vi "labview-quick-extractor.vi"   [LabVIEW 2020]
uses:
  Nominal Client/Nominal Client.lvclass/Nominal Client.ctl
  User/User.lvclass
  Nominal Client/Nominal Client.lvclass
  nominal types/workspace/workspace.lvclass
  submodules/reqwest-labview/lv-src/reqwest/reqwest.lvclass
  datasources/s3/s3.lvclass
  C:/sw/labview-client/lv_src/datasources/source/source.lvclass
  C:/sw/labview-client/lv_src/datasources/payload/payload.lvclass
  C:/sw/labview-client/lv_src/datasources/s3/s3.lvclass
  e79185ee-863a-4b48-b269-365b27d9e424.vi
  Nominal Client/ingest_containerized.vi
  Nominal Client/catalog.wait_until_multiple_ingest_complete.vi
  datasources/target/target.lvclass
  datasources/target/create_new.vi
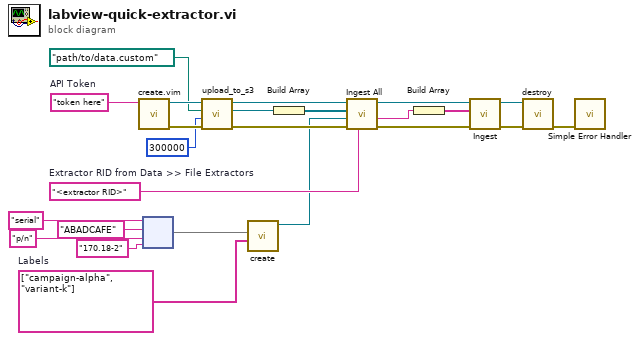
[diagram p0: block diagram]
diagram:
  w2 = string[] ["campaign-alpha", "variant-k"]  # Labels
  w8 = "<extractor RID>"  # Extractor RID from Data >> File Extractors
  w23 = "token here"  # API Token
  n1 = call "create.vim"("API Token (string or path)"=w23) -> ("error out"=w21:errorcluster, "Nominal Client"=w22:refnum<class "Nominal Client.lvclass">)  [unwired: 8 in, 1 out]
  n2 = node("serial", "ABADCAFE", "p/n", "170.18-2") -> (w3:map{string, string})
  n3 = call "upload_to_s3.vi"("error in"=w21, "timeout per chunk (ms)"=300000 ("timeout (ms)"), "File"=path "path/to/data.custom" ("File Path"), "Nominal Client in"=w22) -> ("error out"=w17:errorcluster, "source"=w16:refnum<class "s3.lvclass">, "Nominal Client out"=w18:refnum<class "Nominal Client.lvclass">)  [unwired: 5 in]
  n4 = call-poly "create.vi"("Labels"=w2, "Properties"=w3) -> ("New Target"=w1:refnum<class "target.lvclass">)  [unwired: 9 in]
  n5 = Build Array(w16) -> (w15:refnum<class "s3.lvclass">[])
  n6 = call-poly "Ingest All.vi"("extractorRid"=w8, "error in"=w17, "Target"=w1, "sources"=w15, "Nominal Client in"=w18) -> ("error out"=w11:errorcluster, "datasetRid"=w14:string, "Nominal Client out"=w10:refnum<class "Nominal Client.lvclass">)  [unwired: 3 in, 1 out]
  n7 = Build Array(w14) -> (w9:string[])
  n8 = call-poly "Ingest.vi"("error in"=w11, "datasetRid"=w9, "Nominal Client"=w10) -> ("error out"=w12:errorcluster, "Nominal Client out"=w13:refnum<class "Nominal Client.lvclass">)  [unwired: 7 in]
  n9 = call "destroy.vi"("error in"=w12, "Nominal Client"=w13) -> ("error out"=w24:errorcluster)  [unwired: 9 in]
  n10 = call <vilib>:"Simple Error Handler.vi"("error in (no error)"=w24) -> ()  [unwired: 4 in, 5 out]
